vi "Test Experiment Error Policy.vi"() -> ()   [LabVIEW 2019, in "Transport.lvclass"]
uses:
  Transport.lvclass
panel:
  out "path":path
  out "test ok?":bool[](array[boolean])
  out "text":string
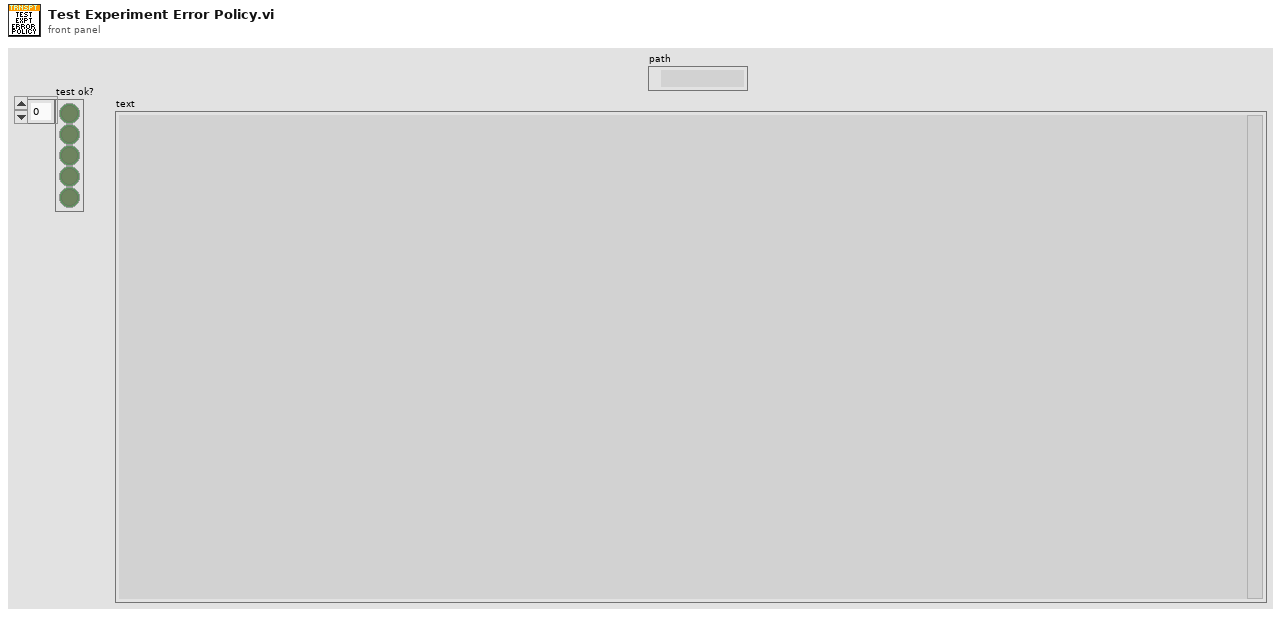
[diagram p1: front panel]
types:
  T1 = cluster{"COM error?":bool, "unhandled error":errorcluster}[]
  T2 = enum16{"open", "replace", "create", "open or create", "replace or create", "replace or create with confirmation"}
  T3 = cluster{"COM error?":bool, "unhandled error":errorcluster}
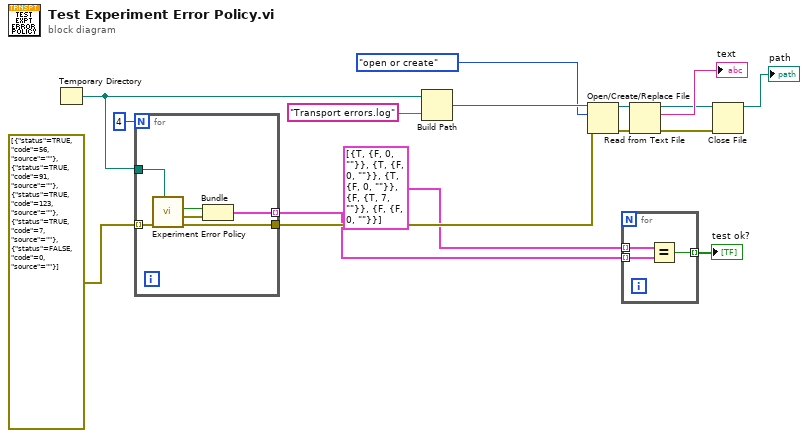
[diagram p0: block diagram]
diagram:
  n1 = Temporary Directory() -> (w15:path)
  n2 = for {
    N: 4 -> [_]
    tunnel: errorcluster[] [{"status"=TRUE, "code"=56, "source"=""}, {"status"=TRUE, "code"=91, "source"=""}, {"status"=TRUE, "code"=123, "source"=""}, {"status"=TRUE, "code"=7, "source"=""}, {"status"=FALSE, "code"=0, "source"=""}] ("error in (no error)") -> [w22] mode=indexing
    tunnel: [w19] -> w4 mode=indexing
    tunnel: w15 -> [w18]
    tunnel: [w17] -> w6
    n3 = call "Experiment Error Policy.vi"("Path"=w18, "error in (no error)"=w22) -> ("handling error"=w17:errorcluster, "unhandled error"=w20:errorcluster, "COM error?"=w21:bool)  [unwired: 6 in, 1 out]
    n4 = Bundle("COM error?"=w21, "unhandled error"=w20) -> (w19:T3)  [unwired: 1 in]
  }
  n5 = Build Path(base path=w15, name or relative path="Transport errors.log") -> (appended path=w11:path)
  n6 = Open/Create/Replace File(file path (use dialog)=w11, error in=w6, operation (0:open)=T2."open or create") -> (refnum out=w9:refnum<file>, error out=w12:errorcluster)  [unwired: 3 in, 1 out]
  n7 = for {
    tunnel: T1 [{"COM error?"=TRUE, "unhandled error"={"status"=FALSE, "code"=0, "source"=""}}, {"COM error?"=TRUE, "unhandled error"={"status"=FALSE, "code"=0, "source"=""}}, {"COM error?"=TRUE, "unhandled error"={"status"=FALSE, "code"=0, "source"=""}}, {"COM error?"=FALSE, "unhandled error"={"status"=TRUE, "code"=7, "source"=""}}, {"COM error?"=FALSE, "unhandled error"={"status"=FALSE, "code"=0, "source"=""}}] ("Array") -> [w25] mode=indexing
    tunnel: w4 -> [w24] mode=indexing
    tunnel: [w23] -> w3 mode=indexing
    n8 = Equal?(x=w25, y=w24) -> (x = y?=w23:bool)
  }
  "test ok?" <- w3
  n9 = Read from Text File(file (use dialog)=w9, error in=w12) -> (refnum out=w8:refnum<file>, text=→"text":string, error out=w7:errorcluster)  [unwired: 2 in, 1 out]
  n10 = Close File(refnum=w8, error in=w7) -> (path=→"path":path)  [unwired: 1 out]
